vi "Read Analog Input and Control Config.vi"() -> (3 "daq cluster":T1)   [LabVIEW 2021]
uses:
  DAQNav Cluster.ctl
  Analog Cluster.ctl
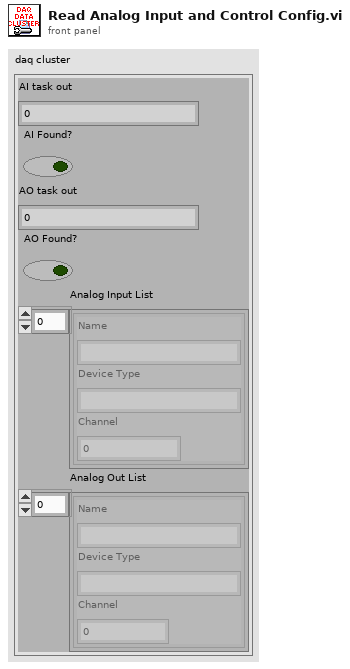
[diagram p1: front panel]
types:
  T1 = typedef "DAQNav Cluster.ctl" = cluster{"AI task out":i32, "AI Found?":bool, "AO task out":i32, "AO Found?":bool, "Analog Input List":T2[], "Analog Out List":T2[]}
  T2 = typedef "Analog Cluster.ctl" = cluster{"Name":string, "Device Type":string, "Channel":i32}
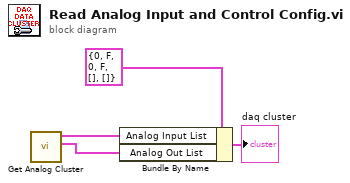
[diagram p0: block diagram]
diagram:
  n1 = call "Get Analog Cluster.vi"() -> ("Analog Output List"=w2:T2[], "Analog Input List"=w3:T2[])  [unwired: 10 in]
  n2 = Bundle By Name(cluster=T1 {"AI task out"=0, "AI Found?"=FALSE, "AO task out"=0, "AO Found?"=FALSE, "Analog Input List"=[], "Analog Out List"=[]} ("Devices.DAQ Device"), "Analog Input List"=w3, "Analog Out List"=w2) -> (→"daq cluster":T1)
